vi "Mast Position Test by Name.vi"() -> ()   [LabVIEW 2023, in "Turn Table and Mast.lvlib" / "CO3000.lvclass"]
uses:
  CO3000.lvclass
  CO3000.lvclass/CO3000.ctl
panel:
  in  "장비Index (-1)":i32=-1
  out "현재 높이 (CH)":dbl
  out "에러 출력":errorcluster
  out "VISA 리소스 이름 출력":refnum<visa-resource-name>
  in  "에러 상수 입력":errorcluster caption="에러 입력(에러 없음)"
  in  "VISA 리소스 이름":refnum<visa-resource-name>
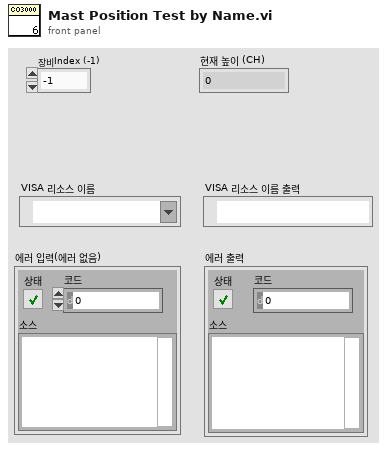
[diagram p1: front panel]
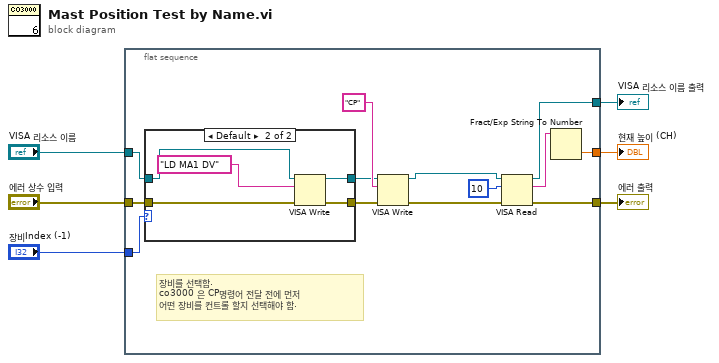
[diagram p0: block diagram]
diagram:
  n1 = flat-sequence {
    tunnel: "에러 상수 입력" -> [w11]
    tunnel: "VISA 리소스 이름" -> [w10]
    tunnel: [w16] -> w4
    tunnel: [w15] -> w3
    tunnel: [w13] -> w2
    tunnel: "장비Index (-1)" -> [w7]
    frame #0 {
      # "장비를 선택함.\nco3000 은 CP명령어 전달 전에 먼저\n어떤 장비를 컨트롤 할지 선택해야 함."
      n2 = case shown="Default" w7 {
        tunnel: w11 -> [w21 w26]
        tunnel: w10 -> [w20 w25]
        tunnel: [w20 w24] -> w9
        tunnel: [w21 w23] -> w8
        frame -1 {
        }
        frame Default {
          n3 = VISA Write(VISA resource name=w25, write buffer="LD MA1 DV" ("버퍼 쓰기"), error in (no error)=w26) -> (VISA resource name out=w24:refnum<visa-resource-name>, error out=w23:errorcluster)  [unwired: 1 out]
        }
      }
      n4 = VISA Write(VISA resource name=w9, write buffer="CP" ("버퍼 쓰기"), error in (no error)=w8) -> (VISA resource name out=w17:refnum<visa-resource-name>, error out=w18:errorcluster)  [unwired: 1 out]
      n5 = VISA Read(VISA resource name=w17, byte count=u32 10 ("바이트 카운트"), error in (no error)=w18) -> (VISA resource name out=w16:refnum<visa-resource-name>, read buffer=w14:string, error out=w15:errorcluster)  [unwired: 1 out]
      n6 = Fract/Exp String To Number(string=w14) -> (number=w13:dbl)  [unwired: 3 in, 1 out]
    }
  }
  "VISA 리소스 이름 출력" <- w4
  "에러 출력" <- w3
  "현재 높이 (CH)" <- w2
